vi "update MultiColumn Listbox Items.vi"(7 "Interpret as Unicode (T)":bool=TRUE, 8 "error in (no error)":errorcluster, 10 "Data[]":string[][](array[string]), 11 "Multicolumn Listbox Ref":refnum<vi>) -> (0 "error out":errorcluster, 3 "Multicolumn Listbox Ref":refnum<vi>)   [LabVIEW 2019, in "Language Selection.lvlib"]
doc: "Uses \"Data[]\" input array to translate a MulticolumListbox control items.\n- - -\nCopyright (c) 2026, Merecs Engineering GmbH"
uses:
  Language Selection.lvlib
panel:
  # "Connector Pane"
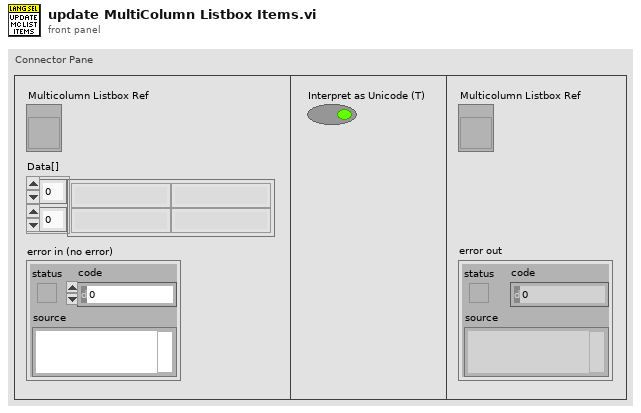
[diagram p1: front panel]
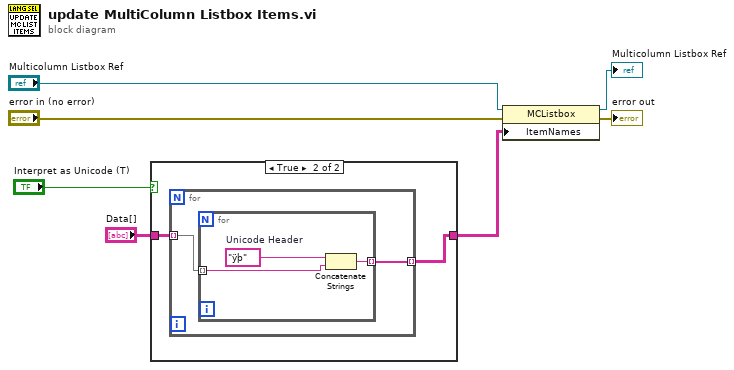
[diagram p0: block diagram]
diagram:
  n1 = case shown="True" "Interpret as Unicode (T)" {
    tunnel: "Data[]" -> [w8 w10]
    tunnel: [w8 w9] -> w6
    frame False {
    }
    frame True {
      n2 = for {
        tunnel: w10 -> [w12] mode=indexing
        tunnel: [w11] -> w9 mode=indexing
        n3 = for {
          tunnel: w12 -> [w15] mode=indexing
          tunnel: [w14] -> w11 mode=indexing
          w13 = "ÿþ"  # Unicode Header
          n4 = Concatenate Strings(w13, w15) -> (w14:string)
        }
      }
    }
  }
  n5 = property class="MCListbox"(reference="Multicolumn Listbox Ref", error in="error in (no error)", "ItemNames"=w6) -> (reference out=→"Multicolumn Listbox Ref":refnum<vi>, error out=→"error out":errorcluster)
